vi "Parse Parameters File.vi"(6 "ch indexing (0-based)":enum16{"0-based", "1-based"}(ring)=enum."1-based", 8 "error in":errorcluster, 11 "path to XML document":path caption="path to parameters xml") -> (0 "error out":errorcluster, 1 "ports":T1[](array[typedef]), 3 "path to XML document out":path caption="path to parameters xml")   [LabVIEW 2020, in "ARINC 429 Import.lvlib"]
uses:
  ARINC 429 Import.lvlib
  <vilib>/xml/NI_XML.lvlib
  <resource>/objmgr/DOMUserDefRef.rc
  <vilib>/NI/NI VeriStand Encoding and Decoding/Encoding.ctl
  <vilib>/NI/NI VeriStand Encoding and Decoding/Encoding and Decoding.lvlib
  Shared/Parameter Definition.ctl
  Shared/Direction.ctl
  Shared/VS Channel Definition for Parameter.ctl
  Shared/VS Channels Definition for Label.ctl
  Shared/VS Channels Definition for All Labels on Hardware Channel.ctl
  Shared/Transfer Type.ctl
  Read Tag Element (U16).vi
  Shared/Transfer Speed.ctl
  <vilib>/xml/Load XML File.vi
  Read Tag Element (Speed).vi
  Read Tag Element (Direction).vi
panel:
  out "parse errors":string
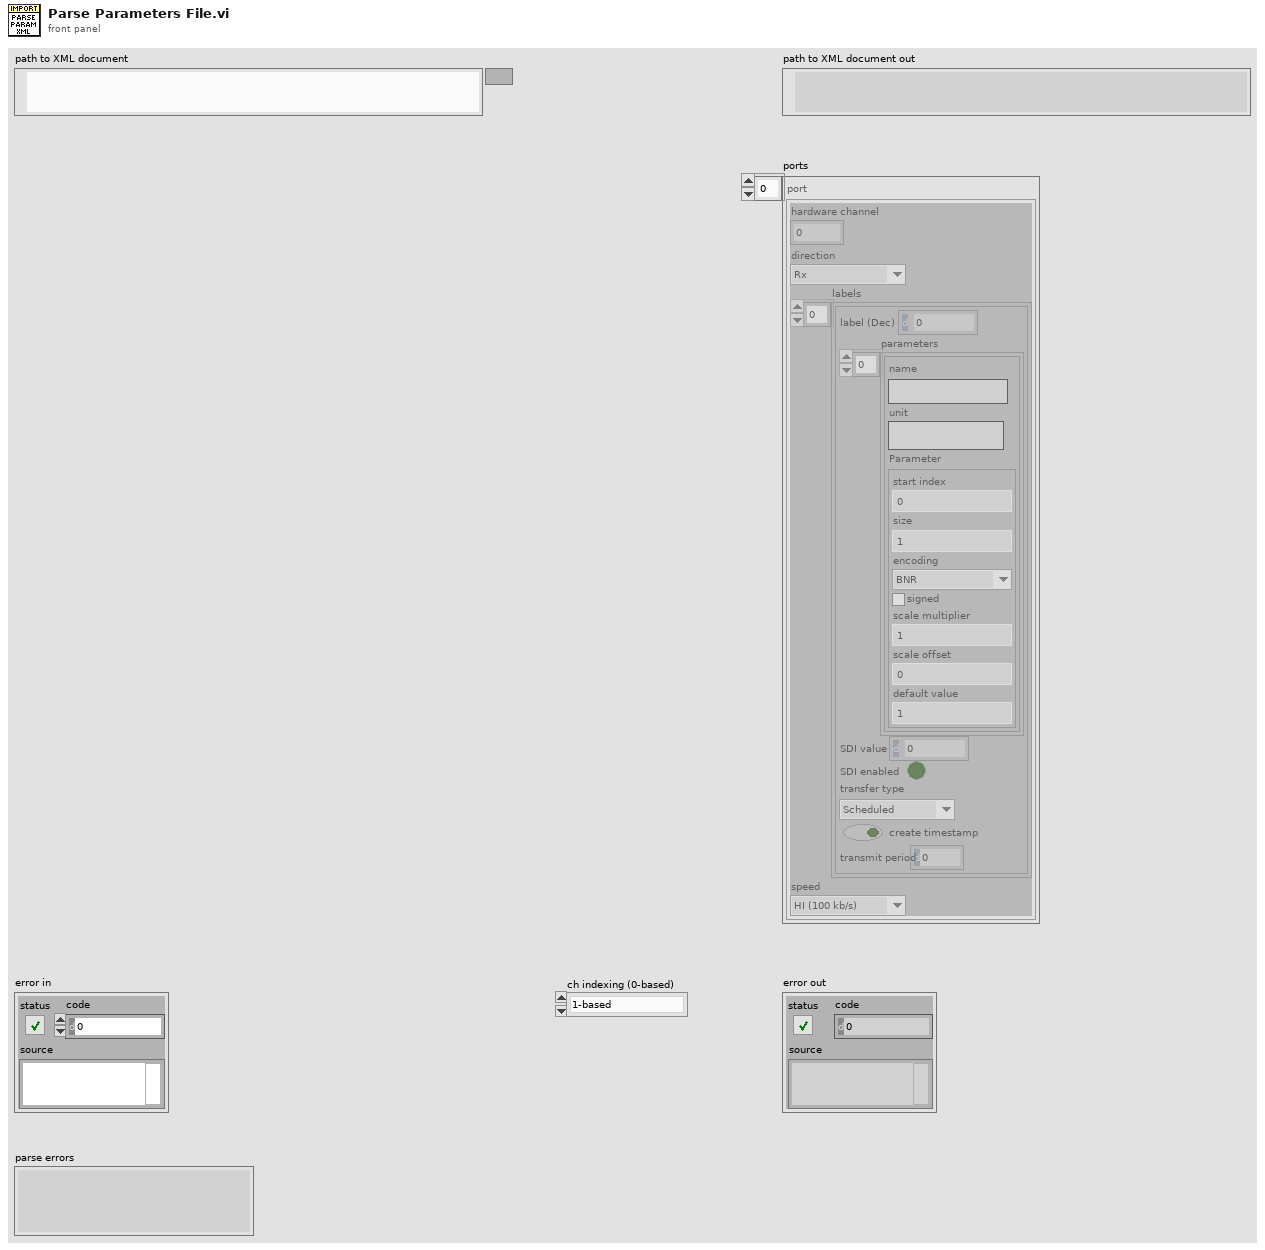
[diagram p1: front panel]
types:
  T1 = typedef "VS Channels Definition for All Labels on Hardware Channel.ctl" = cluster{"hardware channel":i32, "direction":T2, "labels":T3[], "speed":T8}
  T2 = typedef "Direction.ctl" = enum16{"Rx", "Tx"}
  T3 = typedef "VS Channels Definition for Label.ctl" = cluster{"label (Dec)":u32, "parameters":T4[], "SDI value":u8, "SDI enabled":bool, "transfer type":T7, "create timestamp":bool, "transmit period":u32}
  T4 = typedef "VS Channel Definition for Parameter.ctl" = cluster{"name":string, "unit":string, "Parameter":T5}
  T5 = typedef "Parameter Definition.ctl" = cluster{"start index":i32, "size":i32, "encoding":T6, "signed":bool, "scale multiplier":dbl, "scale offset":dbl, "default value":dbl}
  T6 = typedef "Encoding and Decoding.lvlib/Encoding.ctl" = enum16{"BNR", "BCD", "Discrete"}
  T7 = typedef "Transfer Type.ctl" = enum16{"Scheduled", "Acyclic", "Block", "Strobe"}
  T8 = typedef "Transfer Speed.ctl" = enum16{"LO (12.5 kb/s)", "HI (100 kb/s)"}
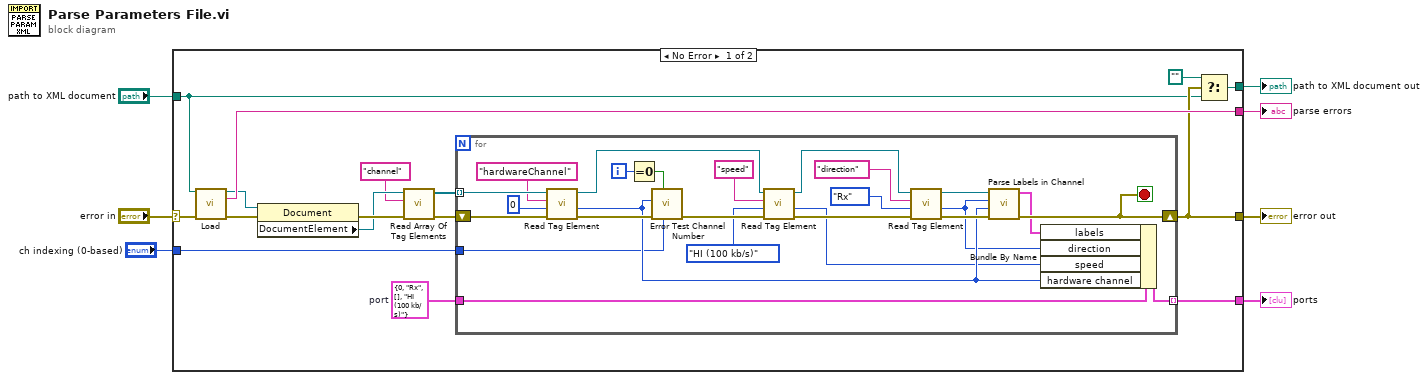
[diagram p0: block diagram]
diagram:
  n1 = case shown="No Error" "error in" {
    selector: "error in" -> [w14 w49]
    tunnel: [w23 _] -> w7
    tunnel: [w21 _] -> w6
    tunnel: [w13 w49] -> w5
    tunnel: "path to XML document" -> [w11 _]
    tunnel: [w12 _] -> w2
    tunnel: "ch indexing (0-based)" -> [w8 _]
    frame No Error {
      w9 = T1 {"hardware channel"=0, "direction"=enum."Rx", "labels"=[], "speed"=enum."HI (100 kb/s)"}  # port
      n2 = call-poly <vilib>:"Load.vi"("path to XML document"=w11, "error in (no error)"=w14) -> ("DOM document out"=w22:refnum<k20>, "parse errors"=w23:string, "error out"=w20:errorcluster)  [unwired: 11 in]
      n3 = property class="Document"(reference=w22, error in=w20) -> (error out=w18:errorcluster, "DocumentElement"=w17:refnum<k20>)  [unwired: 1 out]
      n4 = call "Read Array Of Tag Elements.vi"("error in"=w18, "tag name"="channel" ("Tag Name"), "node in"=w17) -> ("error out"=w19:errorcluster, "array of elements"=w16:refnum<k20>[])  [unwired: 7 in]
      n5 = for {
        tunnel: w16 -> [w48] mode=indexing
        shift-right: [w39] -> w13
        shift-left: w19 -> [w45]
        tunnel: [w47] -> w21 mode=indexing
        tunnel: w9 -> [w34]
        tunnel: w8 -> [w24]
        i -> [w36]
        stop <- w39 stop-if-true
        n6 = call-poly "Read Tag Element.vi"("error in"=w45, "default"=u16 0, "Tag Name"="hardwareChannel", "node in"=w48) -> ("error out"=w42:errorcluster, "value"=w37:u16, "node out"=w32:refnum<k20>)  [unwired: 5 in]
        n7 = Equal To 0?(x=w36) -> (x = 0?=w35:bool)
        n8 = call "Error Test Channel Number.vi"("indexing (0-based)"=w24, "reset (F)"=w35, "error in"=w42, "channel #"=w37) -> ("error out"=w33:errorcluster)  [unwired: 7 in]
        n9 = call-poly "Read Tag Element.vi"("error in"=w33, "default"=Transfer_Speed."HI (100 kb/s)", "Tag Name"="speed", "node in"=w32) -> ("error out"=w30:errorcluster, "value"=w25:T8, "node out"=w31:refnum<k20>)  [unwired: 5 in]
        n10 = call-poly "Read Tag Element.vi"("error in"=w30, "default"=Direction."Rx", "Tag Name"="direction", "node in"=w31) -> ("error out"=w41:errorcluster, "value"=w26:T2, "node out"=w40:refnum<k20>)  [unwired: 5 in]
        n11 = call "Parse Labels in Channel.vi"("error in"=w41, "channel #"=w37, "direction"=w26, "node in"=w40) -> ("error out"=w39:errorcluster, "labels"=w27:T3[])  [unwired: 6 in]
        n12 = Bundle By Name(cluster=w34, "labels"=w27, "direction"=w26, "speed"=w25, "hardware channel"=w37) -> (w47:T1)
      }
      n13 = Select(t=path "", s=w13, f=w11) -> (s? t:f=w12:path)
    }
    frame Error {
    }
  }
  "parse errors" <- w7
  "ports" <- w6
  "error out" <- w5
  "path to XML document out" <- w2
